vi "BB Writer to Refnum.vi"(3 "BB Writer U64":u64) -> (5 "BB Writer Refnum":T1 {"refnum" format="%.0x"})   [LabVIEW 2021, in "Iceoryx.lvlib"]
uses:
  Iceoryx.lvlib
  Typedef/BB Writer Refnum.ctl
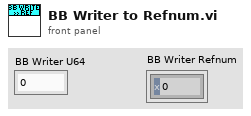
[diagram p1: front panel]
types:
  T1 = typedef "Iceoryx.lvlib/BB Writer Refnum.ctl" = cluster{"refnum":u64, "BB Writer":enum8{"bb_writer"}}
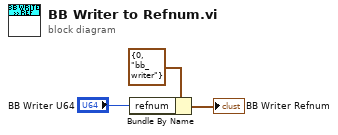
[diagram p0: block diagram]
diagram:
  n1 = Bundle By Name(cluster=T1 {"refnum"=0, "BB Writer"=enum."bb_writer"} ("BB Writer Refnum"), "refnum"="BB Writer U64") -> (→"BB Writer Refnum":T1)
